vi "W12_History.vi"() -> ()   [LabVIEW 2026]
doc: "Use this template to build a VI to use as a subVI."
panel:
  in  "stop":bool
  out "length":i32
  out "history":dbl[](array[numeric])
  in  "N (keep the last N)":i32
  in  "this reading":dbl
  # "Set N first (e.g. 5). One loop = one reading (every 0.1 s)."
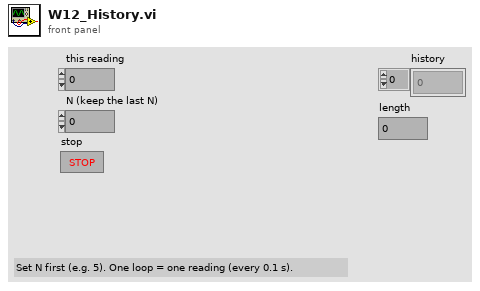
[diagram p1: front panel]
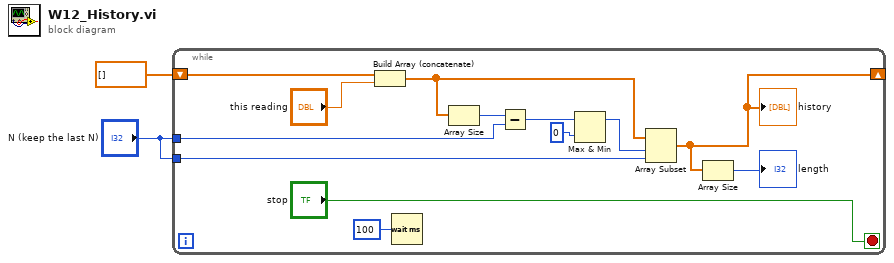
[diagram p0: block diagram]
diagram:
  n1 = while {
    shift-right: [w6] -> _
    shift-left: dbl[] [] -> [w15]
    tunnel: "N (keep the last N)" -> [w11]
    tunnel: "N (keep the last N)" -> [w7]
    stop <- "stop" stop-if-true
    n2 = Build Array (concatenate)(w15, "this reading") -> (w13:dbl[])
    n3 = Wait (ms)(milliseconds to wait=u32 100) -> ()  [unwired: 1 out]
    n4 = Array Size(array=w13) -> (size(s)=w12:i32)
    n5 = Subtract(x=w12, y=w11) -> (x-y=w10:i32)
    n6 = Max & Min(x=w10, y=0) -> (max(x,y)=w8:i32)  [unwired: 1 out]
    n7 = Array Subset(array=w13, index=w8, length=w7) -> (w6:dbl[])
    "history" <- w6
    n8 = Array Size(array=w6) -> (size(s)=→"length":i32)
  }
